vi "Define Test Suite (JUnit Report).vi"(4 "timeout":i32=2000, 5 "register caller level (0)":i32, 6 "Verbose (F)":bool, 8 "error in (no error)":errorcluster, 9 "Report Path":path, 10 "Interactive":bool, 11 "Label (VI Title)":string) -> (0 "error out":errorcluster, 2 "Properties.Suite":refnum<class "Properties.Suite.lvclass">, 3 "Test Suite":refnum<class "Test Suite.lvclass">)   [LabVIEW 2020, in "Caraya.lvlib" / "Test Suite.lvclass"]
doc: "Registers the calling VI as a test suite. If Interactive is True, the interactive user interface is opened when the test suite is executed. If the Report Path is set, a report file will be generated with the test results.\n\n--\nCopyright © 2015 JKI All rights reserved.\n\nAuthor: Tomi Maila <tomi.maila@jki.net>\n\nThis library is provided \"AS IS\" ,WITHOUT WARRANTIES OR\nCONDITIONS OF ANY KIND, either express or implied.\n\nJKI -- jki.net"
uses:
  Test Suite.lvclass
  Properties.Suite/Properties.Suite.lvclass
  C:/projects/caraya/src/classes/Properties/Properties.lvclass
  Test Assert Factory/Test Assert Factory.lvclass
  Test Report.JUnit/Test Report.JUnit.lvclass
  C:/projects/caraya/src/classes/Test Report/Test Report.lvclass
  Test Suite.lvclass/Test Suite.ctl
  Properties.Suite/Properties.Suite.lvclass/Properties.Suite.ctl
  Caraya.lvlib
  Assert Factory Manager/Assert Factory Manager.lvclass
  Basic Test Manager/Basic Test Manager.lvclass
  Properties/Properties.lvclass
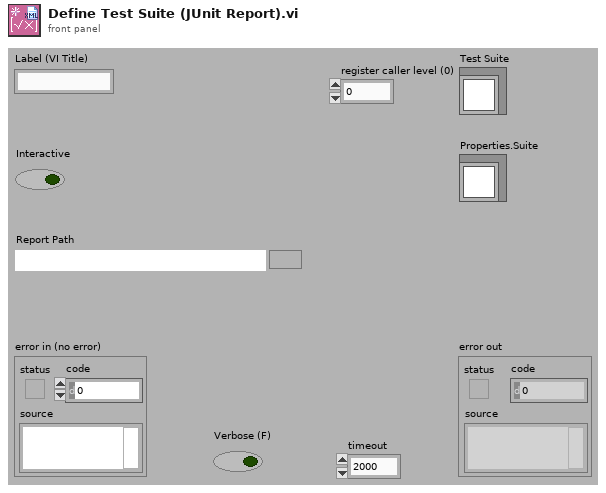
[diagram p1: front panel]
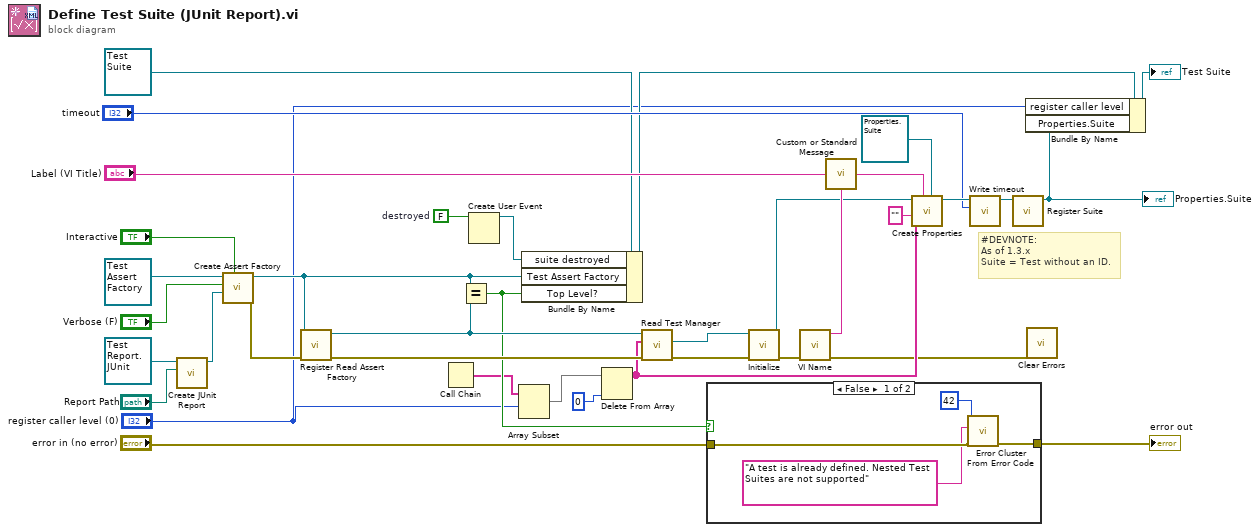
[diagram p0: block diagram]
diagram:
  w18 = FALSE  # destroyed
  # "#DEVNOTE:\nAs of 1.3.x\nSuite = Test without an ID."
  n1 = call "Create JUnit Report.vi"("Report Path"="Report Path", "Test Report.JUnit in"=refnum<class "Test Report.JUnit.lvclass"> refnum) -> ("Test Report.JUnit out"=w24:refnum<class "Test Report.JUnit.lvclass">)  [unwired: 8 in, 1 out]
  n2 = call "Create Assert Factory.vi"("Interactive"="Interactive", "Test Report"=w24, "Verbose (F)"="Verbose (F)", "Test Assert Factory in"=refnum<class "Test Assert Factory.lvclass"> refnum ("Caraya.lvlib:Test Assert Factory.lvclass")) -> ("error out"=w21:errorcluster, "Test Assert Factory out"=w22:refnum<class "Test Assert Factory.lvclass">)  [unwired: 6 in]
  n3 = call "Register Read Assert Factory.vi"("error in (no error)"=w21, "Test Assert Factory"=w22) -> ("error out"=w36:errorcluster, "Test Assert Factory"=w31:refnum<class "Test Assert Factory.lvclass">)  [unwired: 8 in]
  n4 = Call Chain() -> (call chain=w3:string[])
  n5 = Equal?(x=w22, y=w31) -> (x = y?=w19:bool)
  n6 = Create User Event(user event datatype=w18) -> (user event=w17:refnum<user-event>)  [unwired: 1 in, 1 out]
  n7 = Array Subset(array=w3, index="register caller level (0)") -> (w2:string[])  [unwired: 1 in]
  n8 = Bundle By Name(cluster=refnum<class "Test Suite.lvclass"> refnum ("Test Suite"), "suite destroyed"=w17, "Test Assert Factory"=w22, "Top Level?"=w19) -> (w6:refnum<class "Test Suite.lvclass">)
  n9 = Delete From Array(array=w2, index=0) -> (array with subset deleted=w13:string[])  [unwired: 1 in, 1 out]
  n10 = call-dynamic "Read Test Manager.vi"("error in (no error)"=w36, "VI Call Chain"=w13, "Assert Factory in"=w31) -> ("error out"=w34:errorcluster, "Basic Test Manager"=w28:refnum<class "Basic Test Manager.lvclass">)  [unwired: 6 in, 1 out]
  n11 = case shown="False" w19 {
    tunnel: [w41 w42] -> w30
    tunnel: "error in (no error)" -> [w40 w42]
    frame False {
      n12 = call <vilib>:"Error Cluster From Error Code.vi"("error in (no error)"=w40, "error message (\"\")"="A test is already defined. Nested Test Suites are not supported" ("error message (\"\")"), "error code (0)"=42) -> ("error out"=w41:errorcluster)  [unwired: 6 in]
    }
    frame True {
    }
  }
  "error out" <- w30
  n13 = call "Initialize.vi"("error in (no error)"=w34, "Test Manager in"=w28) -> ("error out"=w33:errorcluster, "Test Manager out"=w11:refnum<class "Basic Test Manager.lvclass">)  [unwired: 8 in]
  n14 = call "VI Name.vi"("error in (no error)"=w33) -> ("error out"=w12:errorcluster, "VI Name"=w35:string)  [unwired: 9 in]
  n15 = call "Custom or Standard Message.vi"("Custom Message"="Label (VI Title)", "Standard Message"=w35) -> ("Message"=w14:string)
  n16 = call "Create Properties.vi"("Properties in"=refnum<class "Properties.Suite.lvclass"> refnum ("Caraya.lvlib:Properties.Suite.lvclass"), "label"=w14, "call-chain"=w13, "self-id"="", "Test Manager"=w11) -> ("Properties out"=w10:refnum<class "Properties.Suite.lvclass">)  [unwired: 6 in]
  n17 = call "Write timeout.vi"("timeout"="timeout", "Properties.Suite in"=w10) -> ("Properties.Suite out"=w9:refnum<class "Properties.Suite.lvclass">)  [unwired: 9 in]
  n18 = call "Register Suite.vi"("Properties.Suite in"=w9) -> ("Properties.Suite out"=w4:refnum<class "Properties.Suite.lvclass">)  [unwired: 10 in]
  "Properties.Suite" <- w4
  n19 = Bundle By Name(cluster=w6, "register caller level"="register caller level (0)", "Properties.Suite"=w4) -> (→"Test Suite":refnum<class "Test Suite.lvclass">)
  n20 = call <vilib>:"Clear Errors.vi"("error in (no error)"=w12) -> ()  [unwired: 5 in, 2 out]
